vi "Quick Start - Run - Create.vi"() -> ()   [LabVIEW 2020]
uses:
  Nominal Client/Nominal Client.lvclass/Nominal Client.ctl
  Run/Run.lvclass/Run.ctl
  19192e5f-c46e-4483-8f4d-33940d6cf31d.vi
  Run/rid.get.vi
  Nominal Client/private_data.set.vi
  <vilib>/Utility/file.llb/Application Directory.vi
  <vilib>/Utility/error.llb/Error Cluster From Error Code.vi
  submodules/reqwest-labview/lv-src/reqwest/create.vi
  Nominal Client/Palette Items/who_am_i.vi
  User/User.lvclass
  Nominal Client/Nominal Client.lvclass
  nominal types/workspace/workspace.lvclass
  submodules/reqwest-labview/lv-src/reqwest/reqwest.lvclass
  Run/Run.lvclass
panel:
  in  "Title":string
  out "rid":string
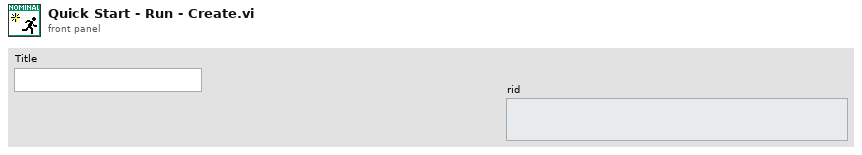
[diagram p1: front panel]
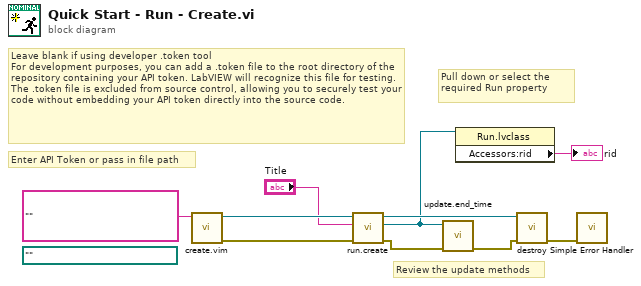
[diagram p0: block diagram]
diagram:
  (unwired) path ""
  # "Review the update methods"
  # "Pull down or select the required Run property"
  # "Leave blank if using developer .token tool\nFor development purposes, you can add a .token file to the root directory of the repository containing your API token. LabVIEW will recognize this file for testing. The .token file is excluded from source control, allowing you to securely test your code without embedding your API token directly into the source code."
  # "Enter API Token or pass in file path"
  n1 = call "create.vim"("API Token (string or path)"="" ("API Token")) -> ("error out"=w8:errorcluster, "Nominal Client"=w9:refnum<class "Nominal Client.lvclass">)  [unwired: 8 in, 1 out]
  n2 = call "run.create.vi"("error in"=w8, "Title"="Title", "Nominal Client in"=w9) -> ("error out"=w1:errorcluster, "Run"=w3:refnum<class "Run.lvclass">, "Nominal Client out"=w7:refnum<class "Nominal Client.lvclass">)  [unwired: 6 in]
  n3 = call "update.end_time.vi"("error in (no error)"=w1, "Run in"=w3) -> ("error out"=w2:errorcluster)  [unwired: 8 in, 1 out]
  n4 = property class="Run.lvclass"(reference=w3) -> ("Accessors:rid"=→"rid":string)  [unwired: 1 in, 2 out]
  n5 = call "destroy.vi"("error in"=w2, "Nominal Client"=w7) -> ("error out"=w6:errorcluster)  [unwired: 9 in]
  n6 = call <vilib>:"Simple Error Handler.vi"("error in (no error)"=w6) -> ()  [unwired: 4 in, 5 out]
